vi "XIS Get Sensor Info.vi"(0 "model":string, 1 "channelType":string, 5 "modelSize":i32, 7 "serialNumber":string, 9 "serialNumberSize":i32, 11 "error in (no error)":errorcluster, 12 "channelTypeSize":i32) -> (3 "channelType out":string, 4 "model out":string, 6 "function return":i32, 8 "serialNumber out":string, 15 "error out":errorcluster)   [LabVIEW 2022 SP3, in "VarexWrapper.lvlib"]
doc: "VAREX_API int XIS_GetSensorInfo(\n char* model, int modelSize,\n char* serialNumber, int serialNumberSize,\n char* channelType, int channelTypeSize);"
uses:
  VarexWrapper.lvlib
  VarexWrapper.dll
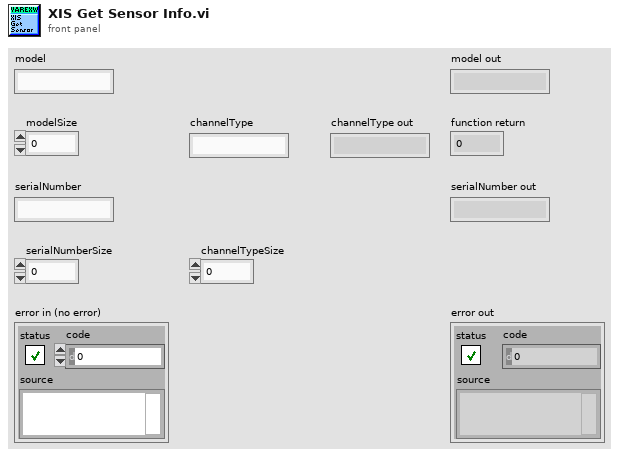
[diagram p1: front panel]
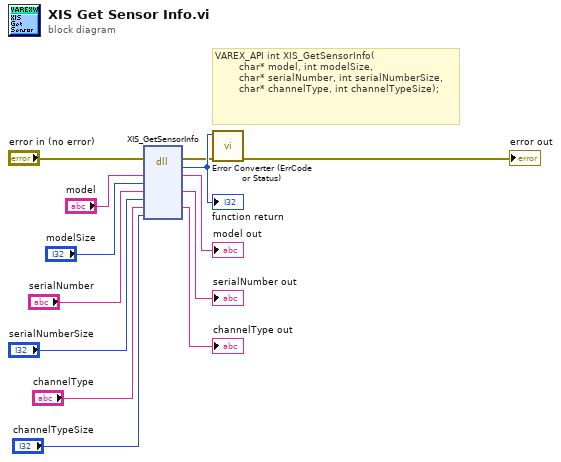
[diagram p0: block diagram]
diagram:
  # "VAREX_API int XIS_GetSensorInfo(\n        char* model, int modelSize,\n        char* serialNumber, int serialNumberSize,\n        char* channelType, int channelTypeSize);"
  n1 = dll-call lib="E:/SourceCodes/image-harvest/ImageHandler/VarexWrapperLvLib/VarexWrapper.*" fn="XIS_GetSensorInfo"(error in="error in (no error)", "model"="model", "modelSize"="modelSize", "serialNumber"="serialNumber", "serialNumberSize"="serialNumberSize", "channelType"="channelType", "channelTypeSize"="channelTypeSize") -> (error out=w2:errorcluster, w13:i32, "model"=→"model out":string, "serialNumber"=→"serialNumber out":string, "channelType"=→"channelType out":string)  [unwired: 5 in, 1 out]
  "function return" <- w13
  n2 = call "Error Converter (ErrCode or Status).vi"("error in (no error)"=w2, "error code"=w13) -> ("error out"=→"error out":errorcluster)  [unwired: 9 in]
